vi "sinewave_and_stop__91854a5d06.vi"(7 "stop steps":i32, 8 "# periods":dbl, 9 "phase":dbl format="%.2p", 10 "amplitude":dbl=1.0 format="%0.2p", 11 "frequency":dbl=10.0 format="%0.2p") -> (0 "expected duration":dbl, 1 "total points":i32, 2 "Waveform Graph":dbl[](graph), 3 "shear points":dbl)   [LabVIEW 2023]
uses:
  <vilib>/Analysis/NI_AALBase.lvlib
panel:
  out "Waveform Graph 2":dbl[](graph)
  out "element":dbl
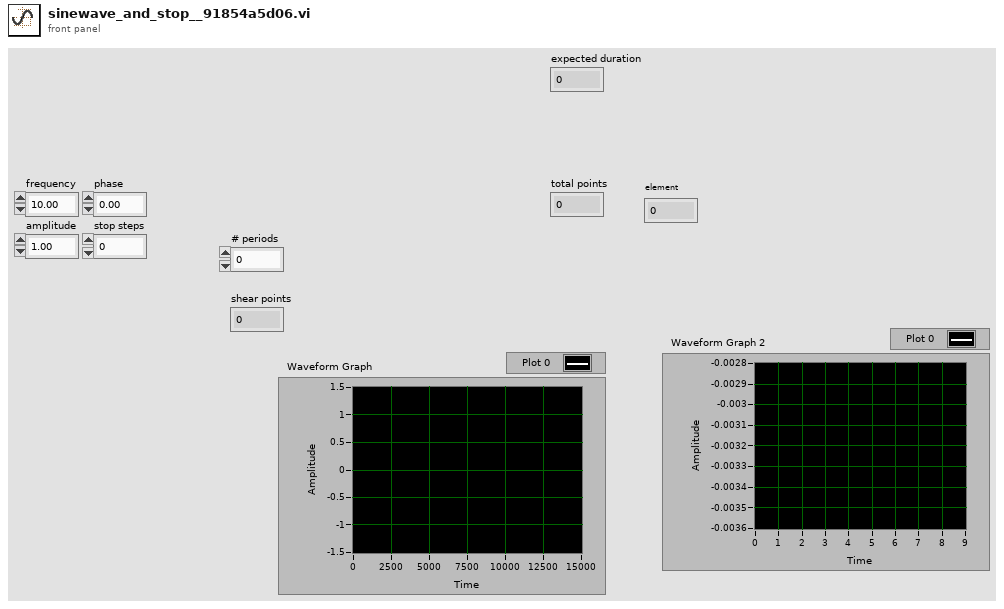
[diagram p1: front panel]
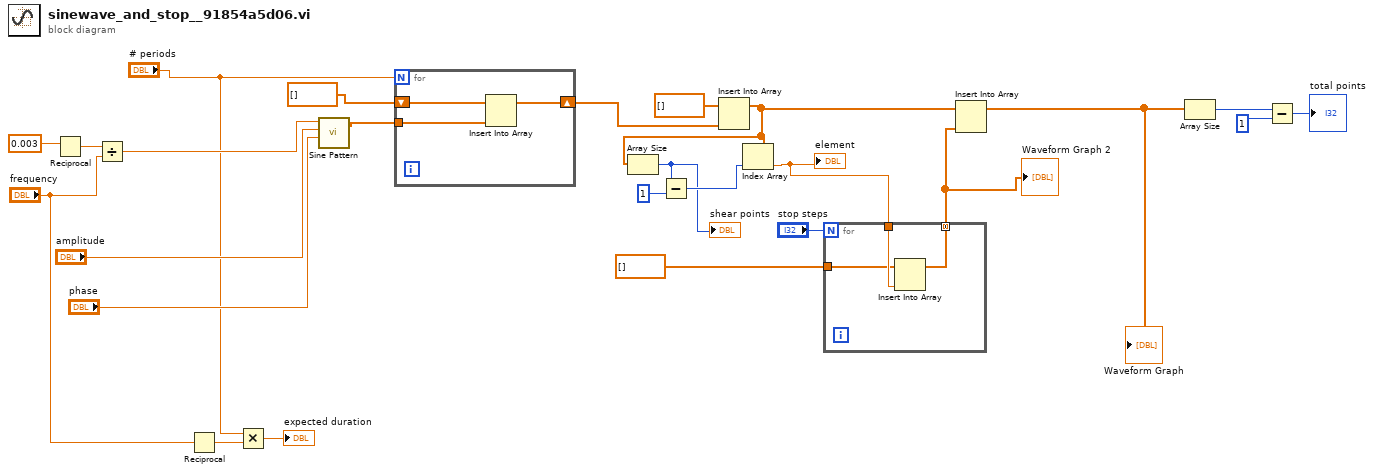
[diagram p0: block diagram]
diagram:
  n1 = Reciprocal(x=0.003) -> (1/x=w15:dbl)
  n2 = Divide(x=w15, y="frequency") -> (x/y=w14:dbl)
  n3 = Reciprocal(x="frequency") -> (1/x=w3:dbl)
  n4 = Multiply(x="# periods", y=w3) -> (x*y=→"expected duration":dbl)
  n5 = call <vilib>:"Sine Pattern.vi"("phase(degrees)"="phase", "amplitude"="amplitude", "samples"=w14) -> ("Sinusoidal Pattern"=w11:dbl[])  [unwired: 1 in, 1 out]
  n6 = for {
    N: "# periods" -> [_]
    tunnel: w11 -> [w28]
    shift-right: [w26] -> w9
    shift-left: dbl[] [] ("array") -> [w27]
    n7 = Insert Into Array(array=w27, new element=w28) -> (w26:dbl[])  [unwired: 1 in]
  }
  n8 = Insert Into Array(array=dbl[] [], new element=w9) -> (w22:dbl[])  [unwired: 1 in]
  n9 = Array Size(array=w22) -> (size(s)=w17:i32)
  "shear points" <- w17
  n10 = Subtract(x=w17, y=1) -> (x-y=w23:i32)
  n11 = Index Array(array=w22, index=w23) -> (element=w20:dbl)
  "element" <- w20
  n12 = for {
    N: "stop steps" -> [_]
    tunnel: w20 -> [w31]
    tunnel: [w30] -> w18 mode=concatenating
    tunnel: dbl[] [] ("array") -> [w29]
    n13 = Insert Into Array(array=w29, new element=w31) -> (w30:dbl[])  [unwired: 1 in]
  }
  "Waveform Graph 2" <- w18
  n14 = Insert Into Array(array=w22, new element=w18) -> (w7:dbl[])  [unwired: 1 in]
  "Waveform Graph" <- w7
  n15 = Array Size(array=w7) -> (size(s)=w6:i32)
  n16 = Subtract(x=w6, y=1) -> (x-y=→"total points":i32)
